vi "Prime BSI R3 Camera Engine.vi"(0 "Prime Notifier Name":string="Not a Name", 11 "Camera Index":string[](array[string])) -> ()   [LabVIEW 2016]
uses:
  Prime BSI Controls/Prime Parameters.ctl
  Prime BSI Controls/Prime Parameter List.ctl
  Prime BSI Controls/Prime ROI.ctl
  Prime BSI Controls/Prime Notifier Element.ctl
  Prime BSI Controls/Prime Actions.ctl
  <vilib>/vision/Image Controls.llb/IMAQ Image.ctl
  Camera Controls/Camera IMAQ Key Info.ctl
  Tools/TIFF Image Read and Write/TIF Write Image Information.ctl
  <vilib>/ptbypt/NI_PtbyPt.lvlib
panel:
  in  "Timing Mode":u32=1
  in  "Set Trigger":bool
  out "mean":dbl format="%0.2f"
  out "Value":dbl format="%.2f"
  in  "Parameter ID":u32
  out "fps":dbl
  out "Image Key Error":errorcluster
  out "Frame":u32
  in  "Init Camera":bool
  in  "Quit":bool
  in  "Use Display Module":bool
  in  "Capture":bool
  in  "Live Preview":bool
  in  "Get ROI":bool
  in  "Set ROI":bool
  in  "Get Parameter":bool
  in  "Set Parameter":bool
  in  "File Save Path":path
  in  "# of Frames":u32
  in  "ROI Setup":T1
  in  "Prime Parameter":T2
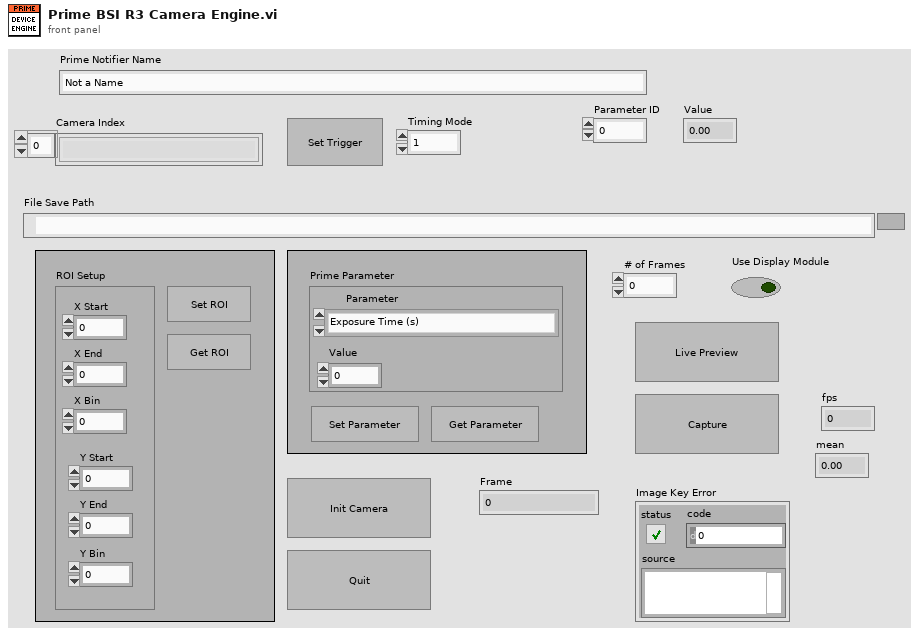
[diagram p1: front panel]
types:
  T1 = typedef "Prime ROI.ctl" = cluster{"X Start":u32, "X End":u32, "X Bin":u32, "Y Start":u32, "Y End":u32, "Y Bin":u32}
  T2 = typedef "Prime Parameters.ctl" = cluster{"Parameter":T3, "Value":dbl}
  T3 = typedef "Prime Parameter List.ctl" = enum16{"Exposure Time (s)"}
  T4 = typedef "Prime Actions.ctl" = enum16{"Error Check", "Initialize", "Preview", "Record", "Abort", "Record Settings", "Set Parameter", "Get Parameter", "Set ROI", "Get ROI", "Status", "Set Trigger", "Quit"}
  T5 = typedef "Image Type" = u32
  T6 = typedef "Prime Notifier Element.ctl" = cluster{"Prime Actions":T4, "Received?":bool, "Prime Parameter":T2, "Prime ROI":T1, "Running?":bool, "File Path":path, "# of frames":u32, "Image Ref":T7, "Error":errorcluster}
  T7 = typedef "IMAQ Image.ctl" = refnum<image>
  T8 = typedef "Camera IMAQ Key Info.ctl" = cluster{"Frame":u32, "Sensor Height":i32, "Sensor Width":i32, "ROI Height":i32, "ROI Width":i32, "ROI Enable?":bool, "Bit per Pixel":u8}
  T9 = enum32{"Invalid", "Standard", "Closed", "Hidden", "Minimized", "Maximized"}
  T10 = typedef "TIF Write Image Information.ctl" = cluster{"Image Width (Pixels)":u32, "Image Height (Pixels)":u32, "Pixel Width (µm)":dbl, "Pixel Height (µm)":dbl, "Bits Per Sample (e.g. 16)":u32, "No. of Frames":u32, "No. of Slices":u32, "Time Step (sec)":dbl, "Z Step (µm)":dbl}
  T11 = enum16{"big-endian, network order", "native, host order", "little-endian"}
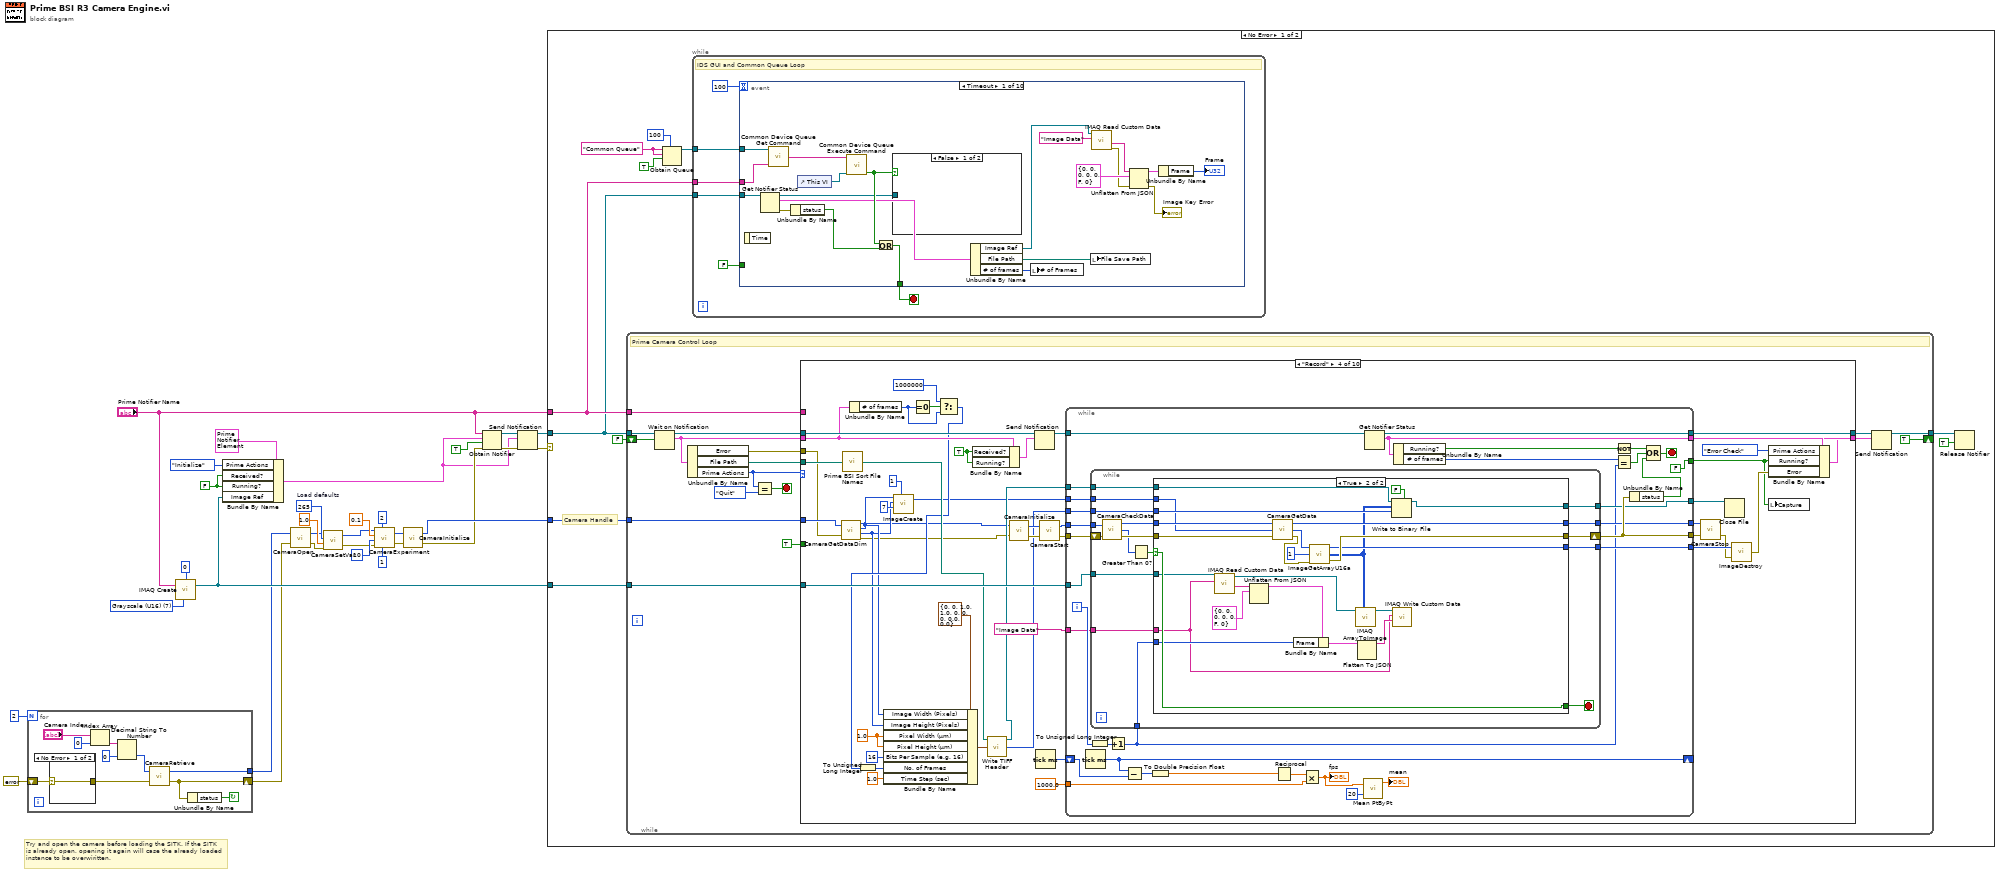
[diagram p0: block diagram]
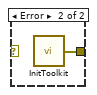
[diagram p2: hidden frame]
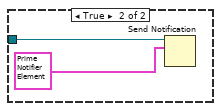
[diagram p3: hidden frame]
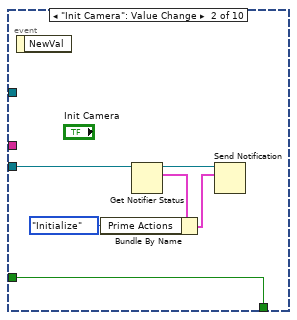
[diagram p4: hidden frame]
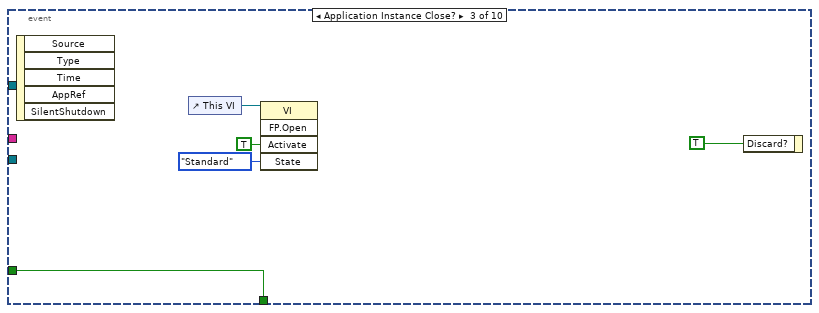
[diagram p5: hidden frame]
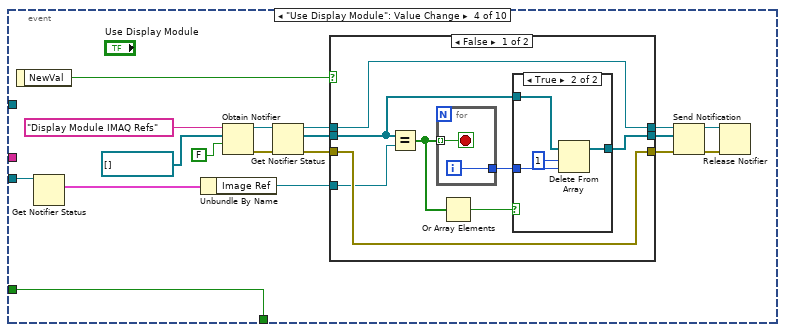
[diagram p6: hidden frame]
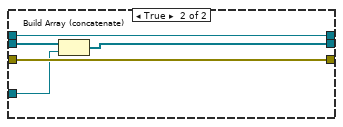
[diagram p8: hidden frame]
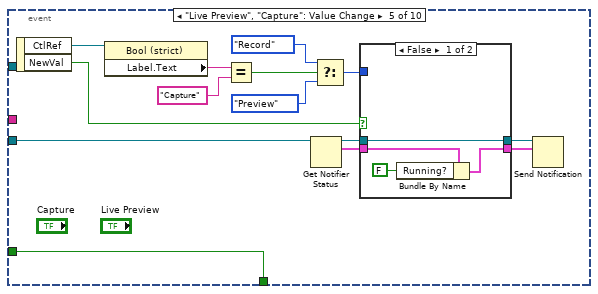
[diagram p9: hidden frame]
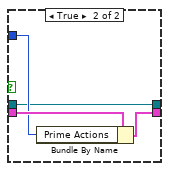
[diagram p10: hidden frame]
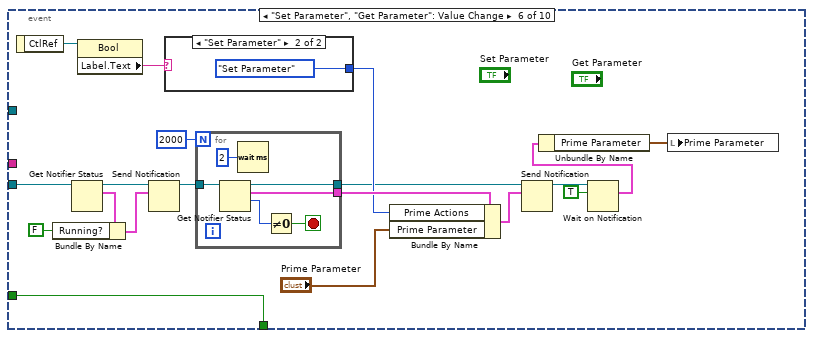
[diagram p11: hidden frame]
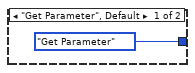
[diagram p12: hidden frame]
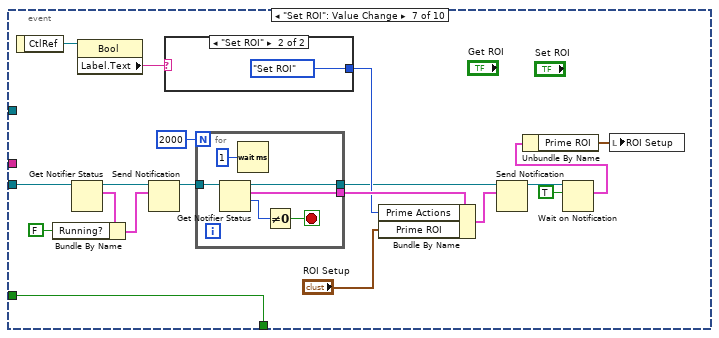
[diagram p13: hidden frame]
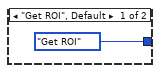
[diagram p14: hidden frame]
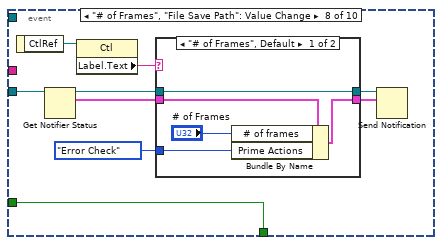
[diagram p15: hidden frame]
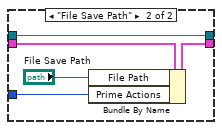
[diagram p16: hidden frame]
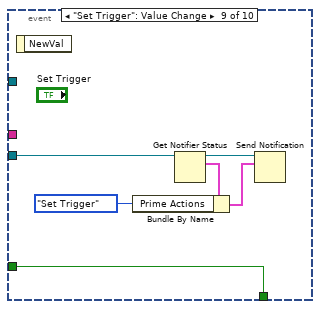
[diagram p17: hidden frame]
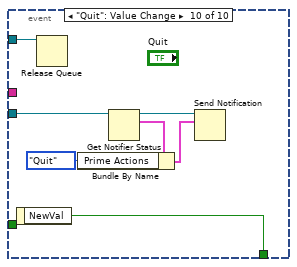
[diagram p18: hidden frame]
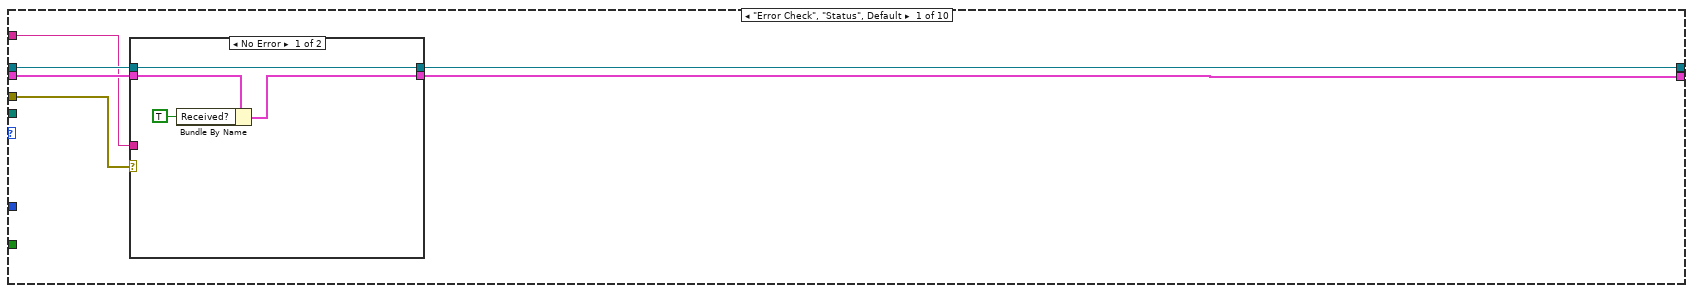
[diagram p19: hidden frame]
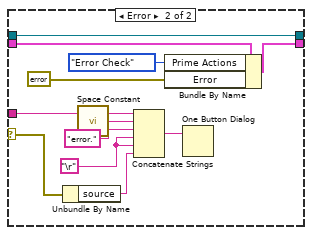
[diagram p20: hidden frame]
diagram:
  w19 = u32 265  # Load defaults
  w21 = FALSE ("Received?")
  w25 = T5 7 items=["Grayscale (U8)", "Grayscale (I16)", "Grayscale (SGL)", "Complex (CSG)", "RGB (U32)", "HSL (U32)", "RGB (U64)", "Grayscale (U16)"] ("Image Type")
  # "Try and open the camera before loading the SITK. If the SITK\nis already open, opening it again will case the already loaded\ninstance to be overwiritten."
  n1 = for {
    N: 2 -> [_]
    tunnel: [w36] -> w13
    shift-right: [w33] -> w12
    shift-left: errorcluster {"status"=FALSE, "code"=0, "source"=""} ("error out") -> [w35]
    stop <- w32 continue-if-true
    n2 = case shown="No Error" w35 {
      selector: w35 -> [w42 _]
      tunnel: [w42 w43] -> w34
      frame No Error {
      }
      frame Error {
        n3 = call <userlib>:"InitToolkit.vi"() -> ("error out"=w43:errorcluster)  [unwired: 1 in]
      }
    }
    n4 = Index Array(array="Camera Index", index=0) -> (element=w39:string)
    n5 = Decimal String To Number(string=w39, default (0L)=u32 0 ("default (0 I32)")) -> (number=w37:u32)  [unwired: 1 in, 1 out]
    n6 = call <userlib>:"CameraRetrieve.vi"("error in"=w34, "Camera Index"=w37) -> ("error out"=w33:errorcluster, "Device ID"=w36:u32)
    n7 = Unbundle By Name(w33) -> ("status"=w32:bool)
  }
  n8 = call "IMAQ Create"("Border Size"=0, "Image Name"="Prime Notifier Name", "Image Type"=w25) -> ("New Image"=w20:T7)  [unwired: 2 in, 1 out]
  n9 = Bundle By Name(cluster=T6 {"Prime Actions"=enum."Initialize", "Received?"=FALSE, "Prime Parameter"={"Parameter"=enum."Exposure Time (s)", "Value"=0.0}, "Prime ROI"={"X Start"=0, "X End"=0, "X Bin"=0, "Y Start"=0, "Y End"=0, "Y Bin"=0}, "Running?"=FALSE, "File Path"=path "", "# of frames"=0, "Image Ref"=refnum, "Error"={"status"=FALSE, "code"=0, "source"=""}} ("IDS Camera Cluster"), "Prime Actions"=Prime_Actions."Initialize" ("IDS Actions"), "Received?"=w21, "Running?"=w21, "Image Ref"=w20) -> (w1:T6)
  n10 = call <userlib>:"CameraOpen.vi"("error in"=w12, "Camera Device ID"=w13) -> ("error out"=w17:errorcluster, "Camera Handle"=w16:u32)
  n11 = call <userlib>:"CameraSetVar.vi"("error in"=w17, "Value"=1.0, "Parameter ID"=w19, "Camera Handle"=w16) -> ("error out"=w4:errorcluster, "CameraHandle"=w5:u32)
  n12 = call <userlib>:"CameraExperiment.vi"("Number of Accumulations"=u32 1, "Acquire / Focus Flag"=u32 2, "error in"=w4, "Number of Images"=u32 10 ("Acquire / Focus Flag"), "Exposure (sec)"=0.1, "Camera Handle"=w5) -> ("error out"=w10:errorcluster, "Camera Handle"=w11:u32)
  n13 = call <userlib>:"CameraInitialize.vi"("error in"=w10, "Camera Handle"=w11) -> ("error out"=w2:errorcluster, "Camera Handle"=w3:u32)
  n14 = Obtain Notifier(name (unnamed)="Prime Notifier Name", notification data type=w1, create if not found? (T)=TRUE, error in (no error)=w2) -> (notifier out=w30:refnum<notifier>, error out=w29:errorcluster)  [unwired: 1 out]
  n15 = Send Notification(notification=w1, notifier=w30, error in (no error)=w29) -> (notifier out=w28:refnum<notifier>, error out=w27:errorcluster)
  n16 = case shown="No Error" w27 {
    selector: w27 -> [_ w616]
    tunnel: w28 -> [w45 w617]
    tunnel: "Prime Notifier Name" -> [w46 w615]
    tunnel: w3 -> [w44 w606]
    tunnel: w20 -> [w52 w609]
    frame No Error {
      w50 = "Common Queue" ("Unique Notifier Name")
      # "Camera Handle"
      n17 = while {
        tunnel: w45 -> [w255]
        tunnel: [w256] -> w53
        tunnel: w44 -> [w249]
        tunnel: w52 -> [w248]
        tunnel: w46 -> [w244]
        shift-right: [TRUE] -> _
        shift-left: FALSE -> [w247]
        stop <- w257 stop-if-true
        # "Prime Camera Control Loop"
        n18 = Wait on Notification(notifier=w255, ignore previous (F)=w247) -> (notifier out=w254:refnum<notifier>, notification=w253:T6)  [unwired: 2 in, 2 out]
        n19 = Unbundle By Name(w253) -> ("Error"=w243:errorcluster, "File Path"=w241:path, "Prime Actions"=w252:T4)
        n20 = Equal?(x=w252, y=Prime_Actions."Quit") -> (x = y?=w257:bool)
        n21 = case shown="\"Record\"" w252 {
          tunnel: w254 -> [w263 w327 w357 w450 w531 w548 w560 w582 w595 w603]
          tunnel: [w262 w327 w336 w435 w531 w548 w560 w582 w595 w603] -> w250
          tunnel: w253 -> [w261 w326 w356 w424 w532 w546 w561 w583 w593 w602]
          tunnel: w244 -> [w260 _ _ _ _ _ _ _ _ _]
          tunnel: w249 -> [_ w313 w351 w445 w535 w543 w577 _ w589 w597]
          tunnel: w248 -> [_ w282 w342 w440 _ _ w564 _ _ w599]
          tunnel: [w259 w324 w355 w449 w538 w549 w579 w585 w591 w600] -> w246
          tunnel: TRUE -> [_ _ _ _ _ _ _ _ _ _]
          tunnel: w243 -> [w258 w281 w329 w405 w536 _ w559 w584 _ _]
          tunnel: w241 -> [_ _ _ w430 _ _ _ _ _ _]
          frame "Error Check", "Status", Default {
            n22 = case shown="No Error" w258 {
              selector: w258 -> [_ w270]
              tunnel: w261 -> [w266 w279]
              tunnel: [w267 w277] -> w262
              tunnel: w263 -> [w267 w277]
              tunnel: w260 -> [_ w276]
              tunnel: [w264 w272] -> w259
              frame No Error {
                n23 = Bundle By Name(cluster=w266, "Received?"=TRUE) -> (w264:T6)
              }
              frame Error {
                w271 = "\r"
                n24 = Unbundle By Name(w270) -> ("source"=w269:string)
                n25 = call <vilib>:"Space Constant.vi"() -> ("String"=w275:string)
                n26 = Concatenate Strings(w276, w275, "error." ("string"), w271, w271, w269) -> (w273:string)
                n27 = Bundle By Name(cluster=w279, "Prime Actions"=Prime_Actions."Error Check" ("IDS Actions"), "Error"=errorcluster {"status"=FALSE, "code"=0, "source"=""}) -> (w272:T6)
                n28 = One Button Dialog(message=w273) -> ()  [unwired: 1 in, 1 out]
              }
            }
          }
          frame "Initialize" {
            w288 = -2  # -2 = fastest adc
            w284 = -1  # -1 = keep what is currently set
            w292 = u32 1 items=["N/A", "Timed Mode/Free run", "Trigger First (only PM)", "Strobed/Ext Sync"] ("Timing Mode")
            w291 = u32 2  # Trigger Edge
            w296 = u32 3  # Shutter State
            w295 = u32 0  # Shutter Comp Time
            w300 = u32 1  # Number of Clears
            w299 = u32 50  # Number of Strips Per Clear
            w301 = u32 0  # Continuous Clears
            w283 = u32 2048 ("X End")
            w305 = u32 1 ("X Start")
            w307 = u32 1  # ROI Number
            w310 = u32 2 items=["Never", "Pre Expos", "Pre Seq", "Post Seq", "Pre-Post Seq", "Pre Expos, Post Seq"] ("Clear Mode")
            w311 = u32 32  # Clear Mode
            w314 = u32 0 items=["First Row", "All Rows", "Any Row", "Max Exposure"] ("Exposure Out")
            w316 = u32 255  # Exposure Out
            n29 = To Double Precision Float(number=w314) -> (double precision float=w315:dbl)
            n30 = call <userlib>:"CameraSetVar.vi"("error in"=w281, "Value"=w315, "Parameter ID"=w316, "Camera Handle"=w313) -> ("error out"=w308:errorcluster, "CameraHandle"=w309:u32)
            n31 = To Double Precision Float(number=w310) -> (double precision float=w312:dbl)
            n32 = Bundle By Name(cluster=T1 {"X Start"=0, "X End"=0, "X Bin"=0, "Y Start"=0, "Y End"=0, "Y Bin"=0} ("ROI Setup"), "X Start"=w305, "X End"=w283, "X Bin"=w305, "Y Start"=w305, "Y End"=w283, "Y Bin"=w305) -> (w304:T1)
            n33 = To Long Integer(number=w283) -> (32bit integer=w280:i32)
            n34 = call <userlib>:"CameraSetVar.vi"("error in"=w308, "Value"=w312, "Parameter ID"=w311, "Camera Handle"=w309) -> ("error out"=w302:errorcluster, "CameraHandle"=w303:u32)
            n35 = call <userlib>:"CameraROI.vi"("error in"=w302, "ROI Params"=w304, "ROI Index"=w307, "Camera Handle"=w303) -> ("error out"=w297:errorcluster, "Camera Handle"=w298:u32)
            n36 = Bundle By Name(cluster=T8 {"Frame"=0, "Sensor Height"=0, "Sensor Width"=0, "ROI Height"=0, "ROI Width"=0, "ROI Enable?"=FALSE, "Bit per Pixel"=0} ("IDS IMAQ Key Info"), "Frame"=u32 0, "Sensor Height"=w280, "Sensor Width"=w280, "ROI Height"=w280, "ROI Width"=w280, "ROI Enable?"=FALSE, "Bit per Pixel"=u8 16) -> (w321:T8)
            n37 = call <userlib>:"CameraCleans.vi"("Camera Handle"=w298, "Number of Clears"=w300, "Number of Strips Per Clear"=w299, "error in"=w297, "Continuous Clears"=w301) -> ("Camera Handle"=w294:u32, "error out"=w293:errorcluster)
            n38 = call <userlib>:"CameraShutter.vi"("Camera Handle"=w294, "Shutter Comp Time: Pre Open"=w295, "Shutter Comp Time: Post Open"=w295, "error in"=w293, "Shutter State"=w296) -> ("Camera Handle"=w290:u32, "error out"=w289:errorcluster)
            n39 = Flatten To JSON(anything=w321) -> (JSON string=w323:string)  [unwired: 2 in, 1 out]
            n40 = call <userlib>:"CameraTrigger.vi"("error in"=w289, "Trigger Edge"=w291, "Timing Mode"=w292, "Camera Handle"=w290) -> ("error out"=w286:errorcluster, "Camera Handle"=w287:u32)
            n41 = call "IMAQ Write Custom Data"("Custom Data In"=w323, "Key"="Image Data", "Image"=w282) -> ()  [unwired: 7 in, 2 out]
            n42 = call <userlib>:"CameraADCset.vi"("ADC offset"=w284, "Read Out port"=w284, "error in (no error)"=w286, "ADC Gain"=w284, "ADC Speed"=w288, "Camera Handle"=w287) -> ("error out"=w285:errorcluster)  [unwired: 1 out]
            n43 = Bundle By Name(cluster=w326, "Prime Actions"=Prime_Actions."Error Check" ("IDS Actions"), "Error"=w285) -> (w324:T6)
          }
          frame "Preview" {
            w333 = FALSE ("Running?")
            w353 = TRUE ("Received?")
            n44 = Bundle By Name(cluster=w356, "Received?"=w353, "Running?"=w353) -> (w354:T6)
            n45 = call <userlib>:"CameraGetDataDim.vi"("Camera Handle"=w351, "error in"=w329) -> ("Camera Handle"=w331:u32, "Xdim"=w350:u32, "Ydim"=w349:u32, "error out"=w346:errorcluster)
            n46 = call <userlib>:"ImageCreate.vi"("X dimension"=w350, "Y dimension"=w349, "Data Type"=u32 7, "error in"=w346, "Number Of Frames"=u32 1) -> ("Image Handle"=w345:u32, "error out"=w330:errorcluster)
            n47 = Send Notification(notification=w354, notifier=w357) -> (notifier out=w341:refnum<notifier>)  [unwired: 1 in, 1 out]
            n48 = call <userlib>:"CameraStart.vi"("error in"=w330, "Camera Handle"=w331) -> ("error out"=w343:errorcluster, "Camera Handle"=w344:u32)
            n49 = while {
              tunnel: w344 -> [w378]
              tunnel: w343 -> [w377]
              tunnel: w345 -> [w374]
              tunnel: w341 -> [w364]
              tunnel: [w363] -> w336
              tunnel: [w366] -> w338
              tunnel: [w376] -> w339
              tunnel: [w375] -> w337
              tunnel: w342 -> [w373]
              tunnel: [w361] -> w335
              shift-right: [w359] -> _
              shift-left: u32 0 ("Frame") -> [w360]
              tunnel: "Image Data" ("Key") -> [w358]
              stop <- w372 stop-if-true
              n50 = call <userlib>:"CameraCheckData.vi"("Camera Handle"=w378, "error in"=w377) -> ("Camera Handle"=w370:u32, "Number Of Frames Available"=w368:i32, "error out"=w371:errorcluster)
              n51 = Greater Than 0?(x=w368) -> (x > 0?=w369:bool)
              n52 = case shown="True" w369 {
                tunnel: w374 -> [w380 w400]
                tunnel: w371 -> [w382 w398]
                tunnel: [w382 w403] -> w366
                tunnel: [w380 w402] -> w375
                tunnel: [w381 w396] -> w376
                tunnel: w370 -> [w381 w399]
                tunnel: w373 -> [_ w386]
                tunnel: w360 -> [w379 w390]
                tunnel: [w379 w389] -> w359
                tunnel: w358 -> [_ w383]
                frame False {
                }
                frame True {
                  n53 = call "IMAQ Read Custom Data"("Key"=w383, "Image"=w386) -> ("Custom Data Out"=w387:string, "Image (duplicate)"=w385:T7)  [unwired: 7 in, 1 out]
                  n54 = Unflatten From JSON(JSON string=w387, type and defaults=T8 {"Frame"=0, "Sensor Height"=0, "Sensor Width"=0, "ROI Height"=0, "ROI Width"=0, "ROI Enable?"=FALSE, "Bit per Pixel"=0} ("IDS IMAQ Key Info")) -> (value=w384:T8)  [unwired: 5 in, 1 out]
                  n55 = Increment(x=w390) -> (x+1=w389:u32)
                  n56 = call <userlib>:"CameraGetData.vi"("error in"=w398, "Image/Data Handle"=w400, "Camera Handle"=w399) -> ("error out"=w395:errorcluster, "Image/Data Handle"=w397:u32, "Camera Handle"=w396:u32)
                  n57 = Bundle By Name(cluster=w384, "Frame"=w389) -> (w392:T8)
                  n58 = call <userlib>:"ImageGetArrayU16a.vi"("error in"=w395, "Z position"=u32 1, "Data Handle"=w397) -> ("error out"=w403:errorcluster, "Array uint 16"=w394:u16[][], "Data Handle"=w402:u32)  [unwired: 1 in]
                  n59 = call "IMAQ ArrayToImage"("Image Pixels (U16)"=w394, "Image"=w385) -> ("Image Out"=w391:T7)  [unwired: 8 in, 1 out]
                  n60 = Flatten To JSON(anything=w392) -> (JSON string=w393:string)  [unwired: 2 in, 1 out]
                  n61 = call "IMAQ Write Custom Data"("Custom Data In"=w393, "Key"=w383, "Image"=w391) -> ()  [unwired: 7 in, 2 out]
                }
              }
              n62 = Get Notifier Status(notifier=w364) -> (notifier out=w363:refnum<notifier>, current notification=w361:T6)  [unwired: 1 in, 3 out]
              n63 = Unbundle By Name(w361) -> ("Running?"=w365:bool)
              n64 = Unbundle By Name(w366) -> ("status"=w367:bool)
              n65 = Not(x=w365) -> (.not. x?=w362:bool)
              n66 = Or(x=w362, y=w367) -> (x .or. y?=w372:bool)
            }
            n67 = call <userlib>:"CameraStop.vi"("error in"=w338, "Camera Handle"=w339) -> ("error out"=w340:errorcluster)  [unwired: 1 out]
            n68 = call <userlib>:"ImageDestroy.vi"("error in"=w340, "Data handle"=w337) -> ("error out"=w334:errorcluster)
            n69 = Bundle By Name(cluster=w335, "Prime Actions"=Prime_Actions."Error Check", "Running?"=w333, "Error"=w334) -> (w355:T6)
            n70 = local write "Capture"(w333) -> ()
          }
          frame "Record" {
            w427 = 1.0 ("Pixel Width (µm)")
            w447 = TRUE ("Received?")
            n71 = call <userlib>:"CameraGetDataDim.vi"("Camera Handle"=w445, "error in"=w405) -> ("Camera Handle"=w407:u32, "Xdim"=w413:u32, "Ydim"=w412:u32, "error out"=w406:errorcluster)
            n72 = call "Prime BSI Sort File Names.vi"("Requested File Path"=w430) -> ("Resulting File Path"=w425:path)  [unwired: 14 in]
            n73 = Unbundle By Name(w424) -> ("# of frames"=w422:u32)
            n74 = call <userlib>:"ImageCreate.vi"("X dimension"=w413, "Y dimension"=w412, "Data Type"=u32 7, "Number Of Frames"=u32 1) -> ("Image Handle"=w411:u32)  [unwired: 1 in, 1 out]
            n75 = Equal To 0?(x=w422) -> (x = 0?=w423:bool)
            n76 = Select(t=u32 1000000, s=w423, f=w422) -> (s? t:f=w420:u32)
            n77 = To Unsigned Long Integer(number=w420) -> (unsigned 32bit integer=w410:u32)
            n78 = Bundle By Name(cluster=T10 {"Image Width (Pixels)"=0, "Image Height (Pixels)"=0, "Pixel Width (µm)"=1.0, "Pixel Height (µm)"=1.0, "Bits Per Sample (e.g. 16)"=0, "No. of Frames"=0, "No. of Slices"=0, "Time Step (sec)"=0.0, "Z Step (µm)"=0.0} ("Image Info"), "Image Width (Pixels)"=w413, "Image Height (Pixels)"=w412, "Pixel Width (µm)"=w427, "Pixel Height (µm)"=w427, "Bits Per Sample (e.g. 16)"=u32 16, "No. of Frames"=w410, "Time Step (sec)"=1.0) -> (w429:T10)
            n79 = Bundle By Name(cluster=w424, "Received?"=w447, "Running?"=w447) -> (w448:T6)
            n80 = call "Write TIFF Header.vi"("File Path"=w425, "Image Info"=w429) -> ("File Ref"=w418:refnum<file>, "Byte Order"=w417:T11)  [unwired: 11 in, 1 out]
            n81 = call <userlib>:"CameraInitialize.vi"("error in"=w406, "Camera Handle"=w407) -> ("error out"=w444:errorcluster, "Camera Handle"=w443:u32)
            n82 = Send Notification(notification=w448, notifier=w450) -> (notifier out=w439:refnum<notifier>)  [unwired: 1 in, 1 out]
            n83 = Tick Count (ms)() -> (millisecond timer value=w432:u32)
            n84 = call <userlib>:"CameraStart.vi"("error in"=w444, "Camera Handle"=w443) -> ("error out"=w441:errorcluster, "Camera Handle"=w442:u32)
            n85 = while {
              tunnel: w442 -> [w483]
              tunnel: w441 -> [w482]
              tunnel: w439 -> [w481]
              tunnel: [w480] -> w435
              tunnel: [w477] -> w437
              tunnel: [w476] -> w438
              tunnel: [w475] -> w436
              tunnel: w440 -> [w473]
              tunnel: [w472] -> w434
              shift-right: [w466] -> _
              shift-left: w432 -> [w467]
              tunnel: 1000.0 -> [w462]
              tunnel: w418 -> [w461]
              tunnel: w417 -> [w460]
              tunnel: [w459] -> w416
              tunnel: w411 -> [w458]
              tunnel: [FALSE ("Running?")] -> w409
              tunnel: "Image Data" ("Key") -> [w451]
              i -> [w470]
              stop <- w478 stop-if-true
              n86 = Tick Count (ms)() -> (millisecond timer value=w466:u32)
              n87 = To Unsigned Long Integer(number=w470) -> (unsigned 32bit integer=w452:u32)
              n88 = Increment(x=w452) -> (x+1=w456:u32)
              n89 = while {
                tunnel: w483 -> [w500]
                tunnel: [w495] -> w476
                tunnel: [w494] -> w475
                tunnel: w473 -> [w491]
                shift-right: [w497] -> w477
                shift-left: w482 -> [w499]
                tunnel: w461 -> [w489]
                tunnel: w460 -> [w488]
                tunnel: [w487] -> w459
                tunnel: w458 -> [w486]
                tunnel: w456 -> [w485]
                tunnel: w451 -> [w484]
                stop <- w490 stop-if-true
                n90 = call <userlib>:"CameraCheckData.vi"("Camera Handle"=w500, "error in"=w499) -> ("Camera Handle"=w496:u32, "Number Of Frames Available"=w493:i32, "error out"=w498:errorcluster)
                n91 = Greater Than 0?(x=w493) -> (x > 0?=w492:bool)
                n92 = case shown="True" w492 {
                  selector: w492 -> [w503 w521]
                  tunnel: w498 -> [w505 w526]
                  tunnel: [w505 w530] -> w497
                  tunnel: [w501 w529] -> w494
                  tunnel: [w504 w525] -> w495
                  tunnel: w496 -> [w504 w527]
                  tunnel: w491 -> [_ w509]
                  tunnel: w485 -> [_ w513]
                  tunnel: [w503 w521] -> w490
                  tunnel: w489 -> [w502 w518]
                  tunnel: w488 -> [_ w517]
                  tunnel: [w502 w515] -> w487
                  tunnel: w486 -> [w501 w514]
                  tunnel: w484 -> [_ w506]
                  frame False {
                  }
                  frame True {
                    n93 = call "IMAQ Read Custom Data"("Key"=w506, "Image"=w509) -> ("Custom Data Out"=w510:string, "Image (duplicate)"=w507:T7)  [unwired: 7 in, 1 out]
                    n94 = Unflatten From JSON(JSON string=w510, type and defaults=T8 {"Frame"=0, "Sensor Height"=0, "Sensor Width"=0, "ROI Height"=0, "ROI Width"=0, "ROI Enable?"=FALSE, "Bit per Pixel"=0} ("IDS IMAQ Key Info")) -> (value=w508:T8)  [unwired: 5 in, 1 out]
                    n95 = call <userlib>:"CameraGetData.vi"("error in"=w526, "Image/Data Handle"=w514, "Camera Handle"=w527) -> ("error out"=w512:errorcluster, "Image/Data Handle"=w520:u32, "Camera Handle"=w525:u32)
                    n96 = Bundle By Name(cluster=w508, "Frame"=w513) -> (w523:T8)
                    n97 = call <userlib>:"ImageGetArrayU16a.vi"("error in"=w512, "Z position"=u32 1, "Data Handle"=w520) -> ("error out"=w530:errorcluster, "Array uint 16"=w516:u16[][], "Data Handle"=w529:u32)  [unwired: 1 in]
                    n98 = call "IMAQ ArrayToImage"("Image Pixels (U16)"=w516, "Image"=w507) -> ("Image Out"=w522:T7)  [unwired: 8 in, 1 out]
                    n99 = Flatten To JSON(anything=w523) -> (JSON string=w524:string)  [unwired: 2 in, 1 out]
                    n100 = Write to Binary File(file (use dialog)=w518, data=w516, 5:FALSE ("prepend array or string size? (T)"), 9:w517) -> (refnum out=w515:refnum<file>)  [unwired: 2 in, 2 out]
                    n101 = call "IMAQ Write Custom Data"("Custom Data In"=w524, "Key"=w506, "Image"=w522) -> ()  [unwired: 7 in, 2 out]
                  }
                }
              }
              n102 = Subtract(x=w466, y=w467) -> (x-y=w465:u32)
              n103 = To Double Precision Float(number=w465) -> (double precision float=w464:dbl)
              n104 = Reciprocal(x=w464) -> (1/x=w463:dbl)
              n105 = Multiply(x=w463, y=w462) -> (x*y=w455:dbl)
              "fps" <- w455
              n106 = call <vilib>:"Mean PtByPt.vi"("x"=w455, "sample length"=20) -> ("mean"=→"mean":dbl)  [unwired: 2 in, 1 out]
              n107 = Get Notifier Status(notifier=w481) -> (notifier out=w480:refnum<notifier>, current notification=w472:T6)  [unwired: 1 in, 3 out]
              n108 = Unbundle By Name(w472) -> ("Running?"=w479:bool, "# of frames"=w471:u32)
              n109 = Not(x=w479) -> (.not. x?=w474:bool)
              n110 = Equal?(x=w471, y=w456) -> (x = y?=w469:bool)
              n111 = Unbundle By Name(w477) -> ("status"=w468:bool)
              n112 = Compound Arithmetic op=OR(w474, w469, w468) -> (w478:bool)
            }
            n113 = call <userlib>:"CameraStop.vi"("error in"=w437, "Camera Handle"=w438) -> ("error out"=w419:errorcluster)  [unwired: 1 out]
            n114 = Close File(refnum=w416) -> ()  [unwired: 1 in, 2 out]
            n115 = call <userlib>:"ImageDestroy.vi"("error in"=w419, "Data handle"=w436) -> ("error out"=w433:errorcluster)
            n116 = Bundle By Name(cluster=w434, "Prime Actions"=Prime_Actions."Error Check", "Running?"=w409, "Error"=w433) -> (w449:T6)
            n117 = local write "Capture"(w409) -> ()
          }
          frame "Get Parameter" {
            n118 = call <userlib>:"CameraGetVar.vi"("Parameter ID"="Parameter ID", "Camera Handle"=w535) -> ("Value"=→"Value":dbl)  [unwired: 1 in, 2 out]
            n119 = Bundle By Name(cluster=w532, "Prime Actions"=Prime_Actions."Error Check" ("IDS Actions"), "Error"=w536, "Received?"=TRUE) -> (w538:T6)
          }
          frame "Set Parameter" {
            n120 = Unbundle By Name(w546) -> ("Prime Parameter.Parameter"=w545:T3, "Prime Parameter.Value"=w544:dbl)
            n121 = case shown="\"Exposure Time (s)\", Default" w545 {
              tunnel: w544 -> [w554]
              tunnel: [w553] -> w542
              tunnel: w543 -> [w552]
              tunnel: [w551] -> w541
              frame "Exposure Time (s)", Default {
                n122 = call <userlib>:"CameraExperiment.vi"("Number of Accumulations"=u32 1, "Acquire / Focus Flag"=u32 2, "Number of Images"=u32 10 ("Acquire / Focus Flag"), "Exposure (sec)"=w554, "Camera Handle"=w552) -> ("error out"=w553:errorcluster, "Camera Handle"=w551:u32)  [unwired: 1 in]
              }
            }
            n123 = call <userlib>:"CameraInitialize.vi"("error in"=w542, "Camera Handle"=w541) -> ("error out"=w540:errorcluster)  [unwired: 1 out]
            n124 = Bundle By Name(cluster=w546, "Prime Actions"=Prime_Actions."Error Check" ("IDS Actions"), "Received?"=TRUE, "Error"=w540) -> (w549:T6)
          }
          frame "Set ROI" {
            w565 = "Image Data" ("Key")
            n125 = Unbundle By Name(w561) -> ("Prime ROI"=w576:T1)
            n126 = call <userlib>:"CameraROI.vi"("error in"=w559, "ROI Params"=w576, "ROI Index"=u32 1, "Camera Handle"=w577) -> ("error out"=w574:errorcluster, "Camera Handle"=w575:u32)
            n127 = call <userlib>:"CameraGetDataDim.vi"("Camera Handle"=w575, "error in"=w574) -> ("Xdim"=w563:u32, "Ydim"=w562:u32, "error out"=w558:errorcluster)  [unwired: 1 out]
            n128 = Bundle By Name(cluster=w561, "Prime Actions"=Prime_Actions."Error Check" ("IDS Actions"), "Error"=w558, "Received?"=TRUE) -> (w579:T6)
            n129 = call "IMAQ Read Custom Data"("Key"=w565, "Image"=w564) -> ("Custom Data Out"=w572:string, "Image (duplicate)"=w573:T7)  [unwired: 7 in, 1 out]
            n130 = To Long Integer(number=w563) -> (32bit integer=w567:i32)
            n131 = To Long Integer(number=w562) -> (32bit integer=w566:i32)
            n132 = Unflatten From JSON(JSON string=w572, type and defaults=T8 {"Frame"=0, "Sensor Height"=0, "Sensor Width"=0, "ROI Height"=0, "ROI Width"=0, "ROI Enable?"=FALSE, "Bit per Pixel"=0} ("IDS IMAQ Key Info")) -> (value=w571:T8)  [unwired: 5 in, 1 out]
            n133 = Bundle By Name(cluster=w571, "ROI Width"=w567, "ROI Height"=w566) -> (w569:T8)
            n134 = Flatten To JSON(anything=w569) -> (JSON string=w568:string)  [unwired: 2 in, 1 out]
            n135 = call "IMAQ Write Custom Data"("Custom Data In"=w568, "Key"=w565, "Image"=w573) -> ()  [unwired: 7 in, 2 out]
          }
          frame "Get ROI" {
            n136 = Bundle By Name(cluster=w583, "Prime Actions"=Prime_Actions."Error Check" ("IDS Actions"), "Error"=w584, "Received?"=TRUE) -> (w585:T6)
          }
          frame "Set Trigger" {
            # "1: Positive Edge\n2: Negative Edge"
            # "Timing Mode\n\n1 = No external trigger (trigger is internal to camera)\n\n2 = External trigger activates all data collection\n\n3 = Each exposure requires a trigger\n\n4 = An external trigger signal controls both the beginning and end of each exposure (Bulb mode). This mode is not valid for all cameras.\n\n5 = External triggers may occur at uneven intervals (Variable mode). This mode is not valid for all cameras.\n\n6 = External trigger activates all data collection (Flash mode). In addition, if the camera is fitted with a flash port, the signal is brought out to these pins. This mode is not valid for all cameras.\n\n7 = Internal trigger. For use when triggering is controlled by a pulse timing generator such as the Princeton Instruments PTG. Note that this mode does not work with older PTG systems."
            n137 = Bundle By Name(cluster=w593, "Prime Actions"=Prime_Actions."Set Trigger", "Received?"=TRUE) -> (w591:T6)
            n138 = call <userlib>:"CameraTrigger.vi"("Trigger Edge"=u32 1, "Timing Mode"="Timing Mode", "Camera Handle"=w589) -> ()  [unwired: 1 in, 2 out]
          }
          frame "Quit" {
            n139 = call "IMAQ Dispose"("Image"=w599) -> ()  [unwired: 5 in, 1 out]
            n140 = call <userlib>:"CameraClose.vi"("Camera Handle"=w597) -> ("error out"=w598:errorcluster)  [unwired: 1 in]
            n141 = call <userlib>:"UninitToolkit.vi"("error in"=w598) -> ("error out"=w596:errorcluster)
            n142 = Bundle By Name(cluster=w602, "Received?"=TRUE, "Error"=w596) -> (w600:T6)
          }
        }
        n143 = Send Notification(notification=w246, notifier=w250) -> (notifier out=w256:refnum<notifier>)  [unwired: 1 in, 1 out]
      }
      n144 = Obtain Queue(max queue size (-1, unlimited)=100, name (unnamed)=w50, element data type=w50, create if not found? (T)=TRUE) -> (queue out=w47:refnum<queue>)  [unwired: 1 in, 2 out]
      n145 = while {
        tunnel: w47 -> [w59]
        tunnel: w46 -> [w57]
        tunnel: w45 -> [w58]
        stop <- w56 stop-if-true
        # "IDS GUI and Common Queue Loop"
        n146 = event shown="[0] Timeout" {
          selector: _ -> [_ _ _ _ _ _ _ _ _ _]
          dyn-events: _ -> [_ _ _ _ _ _ _ _ _ _]
          timeout: 100 -> [_ _ _ _ _ _ _ _ _ _]
          tunnel: w59 -> [w75 _ _ _ _ _ _ _ _ w240]
          tunnel: w58 -> [w74 w88 _ w112 w137 w171 w198 w215 w232 w239]
          tunnel: w57 -> [w73 _ _ _ _ _ _ _ _ _]
          tunnel: [w72 w89 w94 w95 w146 w173 w200 w217 w233 w234] -> w56
          tunnel: FALSE -> [_ w89 w94 w95 w146 w173 w200 w217 w233 _]
          event Timeout {
            n147 = event-data() -> ()  [unwired: 1 in, 1 out]
            n148 = Get Notifier Status(notifier=w74) -> (notifier out=w76:refnum<notifier>, current notification=w69:T6, error out=w81:errorcluster)  [unwired: 1 in, 2 out]
            n149 = call "Common Device Queue Get Command.vi"("Common Queue"=w75, "Notifier Name"=w73) -> ("Command"=w80:string)  [unwired: 12 in, 1 out]
            n150 = Unbundle By Name(w81) -> ("status"=w78:bool)
            n151 = control-ref of="This VI"() -> (w79:refnum<vi>)
            n152 = call "Common Device Queue Execute Command.vi"("Common Command"=w80, "VI Refnum"=w79) -> ("Quit?"=w77:bool)  [unwired: 12 in, 1 out]
            n153 = Or(x=w77, y=w78) -> (x .or. y?=w72:bool)
            n154 = case shown="False" w77 {
              tunnel: w76 -> [_ w83]
              frame False {
              }
              frame True {
                n155 = Send Notification(notification=T6 {"Prime Actions"=enum."Quit", "Received?"=FALSE, "Prime Parameter"={"Parameter"=enum."Exposure Time (s)", "Value"=0.0}, "Prime ROI"={"X Start"=0, "X End"=0, "X Bin"=0, "Y Start"=0, "Y End"=0, "Y Bin"=0}, "Running?"=FALSE, "File Path"=path "", "# of frames"=0, "Image Ref"=refnum, "Error"={"status"=FALSE, "code"=0, "source"=""}} ("IDS Camera Cluster"), notifier=w83) -> ()  [unwired: 1 in, 2 out]
              }
            }
            n156 = Unbundle By Name(w69) -> ("Image Ref"=w67:T7, "File Path"=w71:path, "# of frames"=w70:u32)
            n157 = local write "# of Frames"(w70) -> ()
            n158 = local write "File Save Path"(w71) -> ()
            n159 = call "IMAQ Read Custom Data"("Key"="Image Data", "Image"=w67) -> ("error out"=w62:errorcluster, "Custom Data Out"=w65:string)  [unwired: 7 in, 1 out]
            n160 = Unflatten From JSON(JSON string=w65, type and defaults=T8 {"Frame"=0, "Sensor Height"=0, "Sensor Width"=0, "ROI Height"=0, "ROI Width"=0, "ROI Enable?"=FALSE, "Bit per Pixel"=0} ("IDS IMAQ Key Info"), error in (no error)=w62) -> (value=w64:T8, error out=→"Image Key Error":errorcluster)  [unwired: 4 in]
            n161 = Unbundle By Name(w64) -> ("Frame"=→"Frame":u32)
          }
          event "Init Camera": Value Change {
            n162 = event-data() -> ()  [unwired: 1 in, 1 out]
            n163 = Get Notifier Status(notifier=w88) -> (notifier out=w84:refnum<notifier>, current notification=w87:T6)  [unwired: 1 in, 3 out]
            n164 = Bundle By Name(cluster=w87, "Prime Actions"=Prime_Actions."Initialize" ("IDS Actions")) -> (w85:T6)
            n165 = Send Notification(notification=w85, notifier=w84) -> ()  [unwired: 1 in, 2 out]
          }
          event Application Instance Close? {
            n166 = event-data() -> ()  [unwired: 1 in, 5 out]
            n167 = control-ref of="This VI"() -> (w91:refnum<vi>)
            n168 = invoke class="VI" method="FP.Open"(reference=w91, "Activate"=TRUE ("Activate?"), "State"=T9."Standard") -> ()  [unwired: 2 in, 5 out]
            n169 = event-data("Discard?"=TRUE) -> ()  [unwired: 1 in, 1 out]
          }
          event "Use Display Module": Value Change {
            n170 = event-data() -> ("NewVal"=w97:bool)  [unwired: 1 in]
            n171 = Get Notifier Status(notifier=w112) -> (current notification=w111:T6)  [unwired: 1 in, 4 out]
            n172 = Unbundle By Name(w111) -> ("Image Ref"=w96:T7)
            n173 = Obtain Notifier(name (unnamed)="Display Module IMAQ Refs", notification data type=T7[] [], create if not found? (T)=FALSE) -> (notifier out=w104:refnum<notifier>, error out=w103:errorcluster)  [unwired: 1 in, 1 out]
            n174 = Get Notifier Status(notifier=w104, error in (no error)=w103) -> (notifier out=w105:refnum<notifier>, current notification=w107:T7[], error out=w106:errorcluster)  [unwired: 2 out]
            n175 = case shown="False" w97 {
              tunnel: w105 -> [w120 w130]
              tunnel: w106 -> [w114 w129]
              tunnel: w107 -> [w116 w132]
              tunnel: [w115 w131] -> w110
              tunnel: [w120 w130] -> w108
              tunnel: [w114 w129] -> w109
              tunnel: w96 -> [w113 w128]
              frame False {
                n176 = Equal?(x=w116, y=w113) -> (x = y?=w119:bool[])
                n177 = for {
                  tunnel: w119 -> [w127] mode=indexing
                  tunnel: [w126] -> w117
                  i -> [w126]
                  stop <- w127 stop-if-true
                }
                n178 = Or Array Elements(Boolean array=w119) -> (logical OR=w118:bool)
                n179 = case shown="True" w118 {
                  tunnel: w117 -> [_ w124]
                  tunnel: w116 -> [w121 w123]
                  tunnel: [w121 w122] -> w115
                  frame False {
                  }
                  frame True {
                    n180 = Delete From Array(array=w123, length=1, index=w124) -> (array with subset deleted=w122:T7[])  [unwired: 1 out]
                  }
                }
              }
              frame True {
                n181 = Build Array (concatenate)(w132, w128) -> (w131:T7[])
              }
            }
            n182 = Send Notification(notification=w110, notifier=w108, error in (no error)=w109) -> (notifier out=w102:refnum<notifier>, error out=w101:errorcluster)
            n183 = Release Notifier(notifier=w102, error in (no error)=w101) -> ()  [unwired: 1 in, 3 out]
          }
          event "Live Preview", "Capture": Value Change {
            n184 = event-data() -> ("CtlRef"=w145:refnum<vi>, "NewVal"=w139:bool)  [unwired: 1 in]
            n185 = property class="Bool (strict)"(reference=w145) -> ("Label.Text"=w144:string)  [unwired: 1 in, 2 out]
            n186 = Equal?(x=w144, y="Capture") -> (x = y?=w142:bool)
            n187 = Get Notifier Status(notifier=w137) -> (notifier out=w136:refnum<notifier>, current notification=w135:T6)  [unwired: 1 in, 3 out]
            n188 = Select(t=Prime_Actions."Record" ("y"), s=w142, f=Prime_Actions."Preview" ("y")) -> (s? t:f=w138:T4)
            n189 = case shown="False" w139 {
              tunnel: w138 -> [_ w153]
              tunnel: w136 -> [w148 w152]
              tunnel: w135 -> [w150 w154]
              tunnel: [w148 w152] -> w134
              tunnel: [w147 w151] -> w133
              frame False {
                n190 = Bundle By Name(cluster=w150, "Running?"=FALSE) -> (w147:T6)
              }
              frame True {
                n191 = Bundle By Name(cluster=w154, "Prime Actions"=w153) -> (w151:T6)
              }
            }
            n192 = Send Notification(notification=w133, notifier=w134) -> ()  [unwired: 1 in, 2 out]
          }
          event "Set Parameter", "Get Parameter": Value Change {
            n193 = event-data() -> ("CtlRef"=w172:refnum<vi>)  [unwired: 1 in]
            n194 = Get Notifier Status(notifier=w171) -> (notifier out=w166:refnum<notifier>, current notification=w169:T6)  [unwired: 1 in, 3 out]
            n195 = Bundle By Name(cluster=w169, "Running?"=FALSE) -> (w165:T6)
            n196 = property class="Bool"(reference=w172) -> ("Label.Text"=w170:string)  [unwired: 1 in, 2 out]
            n197 = Send Notification(notification=w165, notifier=w166) -> (notifier out=w164:refnum<notifier>)  [unwired: 1 in, 1 out]
            n198 = case shown="\"Set Parameter\"" w170 {
              tunnel: [Prime_Actions."Get Parameter" ("IDS Actions") Prime_Actions."Set Parameter" ("IDS Actions")] -> w161
              frame "Get Parameter", Default {
              }
              frame "Set Parameter" {
              }
            }
            n199 = for {
              N: 2000 -> [_]
              tunnel: w164 -> [w178]
              tunnel: [w177] -> w160
              tunnel: [w176] -> w163
              stop <- w174 stop-if-true
              n200 = Get Notifier Status(notifier=w178) -> (notifier out=w177:refnum<notifier>, current notification=w176:T6, # waiting=w175:i32)  [unwired: 1 in, 2 out]
              n201 = Wait (ms)(milliseconds to wait=u32 2) -> ()  [unwired: 1 out]
              n202 = Not Equal To 0?(x=w175) -> (x != 0?=w174:bool)
            }
            n203 = Bundle By Name(cluster=w163, "Prime Actions"=w161, "Prime Parameter"="Prime Parameter") -> (w159:T6)
            n204 = Send Notification(notification=w159, notifier=w160) -> (notifier out=w158:refnum<notifier>)  [unwired: 1 in, 1 out]
            n205 = Wait on Notification(notifier=w158, ignore previous (F)=TRUE) -> (notification=w156:T6)  [unwired: 2 in, 3 out]
            n206 = Unbundle By Name(w156) -> ("Prime Parameter"=w155:T2)
            n207 = local write "Prime Parameter"(w155) -> ()
          }
          event "Set ROI": Value Change {
            n208 = event-data() -> ("CtlRef"=w199:refnum<vi>)  [unwired: 1 in]
            n209 = Get Notifier Status(notifier=w198) -> (notifier out=w193:refnum<notifier>, current notification=w196:T6)  [unwired: 1 in, 3 out]
            n210 = Bundle By Name(cluster=w196, "Running?"=FALSE) -> (w192:T6)
            n211 = property class="Bool"(reference=w199) -> ("Label.Text"=w197:string)  [unwired: 1 in, 2 out]
            n212 = Send Notification(notification=w192, notifier=w193) -> (notifier out=w191:refnum<notifier>)  [unwired: 1 in, 1 out]
            n213 = case shown="\"Set ROI\"" w197 {
              tunnel: [Prime_Actions."Get ROI" ("IDS Actions") Prime_Actions."Set ROI" ("IDS Actions")] -> w189
              frame "Get ROI", Default {
              }
              frame "Set ROI" {
              }
            }
            n214 = for {
              N: 2000 -> [_]
              tunnel: w191 -> [w205]
              tunnel: [w204] -> w188
              tunnel: [w203] -> w190
              stop <- w201 stop-if-true
              n215 = Get Notifier Status(notifier=w205) -> (notifier out=w204:refnum<notifier>, current notification=w203:T6, # waiting=w202:i32)  [unwired: 1 in, 2 out]
              n216 = Wait (ms)(milliseconds to wait=u32 1) -> ()  [unwired: 1 out]
              n217 = Not Equal To 0?(x=w202) -> (x != 0?=w201:bool)
            }
            n218 = Bundle By Name(cluster=w190, "Prime Actions"=w189, "Prime ROI"="ROI Setup") -> (w187:T6)
            n219 = Send Notification(notification=w187, notifier=w188) -> (notifier out=w186:refnum<notifier>)  [unwired: 1 in, 1 out]
            n220 = Wait on Notification(notifier=w186, ignore previous (F)=TRUE) -> (notification=w184:T6)  [unwired: 2 in, 3 out]
            n221 = Unbundle By Name(w184) -> ("Prime ROI"=w183:T1)
            n222 = local write "ROI Setup"(w183) -> ()
          }
          event "# of Frames", "File Save Path": Value Change {
            n223 = event-data() -> ("CtlRef"=w216:refnum<vi>)  [unwired: 1 in]
            n224 = Get Notifier Status(notifier=w215) -> (notifier out=w213:refnum<notifier>, current notification=w212:T6)  [unwired: 1 in, 3 out]
            n225 = property class="Ctl"(reference=w216) -> ("Label.Text"=w214:string)  [unwired: 1 in, 2 out]
            n226 = case shown="\"# of Frames\", Default" w214 {
              tunnel: w213 -> [w220 w227]
              tunnel: w212 -> [w222 w226]
              tunnel: [w220 w227] -> w211
              tunnel: [w219 w225] -> w210
              tunnel: Prime_Actions."Error Check" ("IDS Actions") -> [w218 w223]
              frame "# of Frames", Default {
                n227 = Bundle By Name(cluster=w222, "# of frames"="# of Frames", "Prime Actions"=w218) -> (w219:T6)
              }
              frame "File Save Path" {
                n228 = Bundle By Name(cluster=w226, "File Path"="File Save Path", "Prime Actions"=w223) -> (w225:T6)
              }
            }
            n229 = Send Notification(notification=w210, notifier=w211) -> ()  [unwired: 1 in, 2 out]
          }
          event "Set Trigger": Value Change {
            n230 = event-data() -> ()  [unwired: 1 in, 1 out]
            n231 = Get Notifier Status(notifier=w232) -> (notifier out=w231:refnum<notifier>, current notification=w230:T6)  [unwired: 1 in, 3 out]
            n232 = Bundle By Name(cluster=w230, "Prime Actions"=Prime_Actions."Set Trigger") -> (w228:T6)
            n233 = Send Notification(notification=w228, notifier=w231) -> ()  [unwired: 1 in, 2 out]
          }
          event "Quit": Value Change {
            n234 = event-data() -> ("NewVal"=w234:bool)  [unwired: 1 in]
            n235 = Release Queue(queue=w240) -> ()  [unwired: 2 in, 3 out]
            n236 = Get Notifier Status(notifier=w239) -> (notifier out=w238:refnum<notifier>, current notification=w237:T6)  [unwired: 1 in, 3 out]
            n237 = Bundle By Name(cluster=w237, "Prime Actions"=Prime_Actions."Quit" ("IDS Actions")) -> (w235:T6)
            n238 = Send Notification(notification=w235, notifier=w238) -> ()  [unwired: 1 in, 2 out]
          }
        }
      }
      n239 = Release Notifier(notifier=w53, force destroy? (F)=TRUE) -> ()  [unwired: 1 in, 3 out]
    }
    frame Error {
      n240 = Release Notifier(notifier=w617, force destroy? (F)=TRUE, error in (no error)=w616) -> (error out=w605:errorcluster)  [unwired: 2 out]
      n241 = call <userlib>:"CameraClose.vi"("error in"=w605, "Camera Handle"=w606) -> ("error out"=w607:errorcluster)
      n242 = call <userlib>:"UninitToolkit.vi"("error in"=w607) -> ("error out"=w604:errorcluster)
      n243 = call "IMAQ Dispose"("Image"=w609, "error in (no error)"=w604) -> ("error out"=w608:errorcluster)  [unwired: 4 in]
      n244 = Unbundle By Name(w608) -> ("source"=w610:string)
      n245 = call <vilib>:"Space Constant.vi"() -> ("String"=w613:string)
      n246 = Concatenate Strings(w615, w613, "Device Error." ("string"), "\r", w610) -> (w614:string)
      n247 = One Button Dialog(message=w614) -> ()  [unwired: 1 in, 1 out]
    }
  }
